vi "撒旦.vi"(2 "Cluster":cluster{"Numeric":dbl}, 7 "VISA resource name":refnum<visa-resource-name>, 9 "Array":bool[](array[boolean]), 10 "Path":path) -> ()   [LabVIEW 2017]
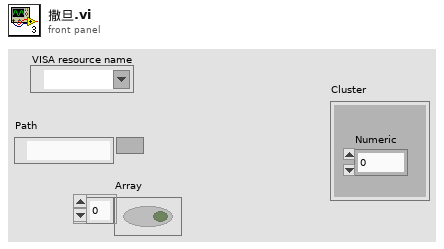
[diagram p1: front panel]
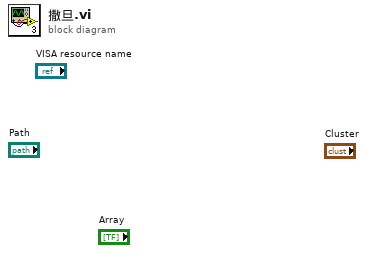
[diagram p0: block diagram]
diagram:
